vi "Game_Play.vi"(0 "State":T1={"Tick"=0, "Phase"=0, "PhaseTicks"=0, "Level"=1, "Room"=0, "X10"=0, "Y10"=0, "VY10"=0, "Mode"=0, "Facing"=0, "Run"=0, "Vert"=0, "StandY"=0, "EntryX10"=0, "EntryY10"=0, "EntryMode"=0, "Lives"=4, "Score"=0, "NextLife"=10000, "KeyR"=0, "KeyB"=0, "KeyY"=0, "Torch"=FALSE, "FloorPhase"=0, "Dead"=FALSE, "LevelStart"=FALSE, "Quit"=FALSE, "Sound"=0, "Seed"=12345, "DemoStep"=0, "Tiles"=[], "World"=[], "Enemies"=[], "Highscores"=[], "Name"=[0, 0, 0], "Cursor"=0}, 5 "Jump":bool, 11 "error in":errorcluster) -> (4 "State out":T1={"Tick"=0, "Phase"=0, "PhaseTicks"=0, "Level"=1, "Room"=0, "X10"=0, "Y10"=0, "VY10"=0, "Mode"=0, "Facing"=0, "Run"=0, "Vert"=0, "StandY"=0, "EntryX10"=0, "EntryY10"=0, "EntryMode"=0, "Lives"=4, "Score"=0, "NextLife"=10000, "KeyR"=0, "KeyB"=0, "KeyY"=0, "Torch"=FALSE, "FloorPhase"=0, "Dead"=FALSE, "LevelStart"=FALSE, "Quit"=FALSE, "Sound"=0, "Seed"=12345, "DemoStep"=0, "Tiles"=[], "World"=[], "Enemies"=[], "Highscores"=[], "Name"=[0, 0, 0], "Cursor"=0}, 6 "Hit":bool, 8 "Died":bool, 15 "error out":errorcluster)   [LabVIEW 2020, in "GH_Engine.lvlib"]
doc: "One tick of play: rhythm of the vanishing floors (FloorPhase), Claude moves (Player_Move, jump sound), takes objects (Items_Collect), opens doors (Door_Open), enemies move (Enemies_Step), Hit_Check, room change (Room_Change) and an extra life every 10000 points (at most 7). Hit = an enemy touches Claude, Died = deadly fall."
uses:
  GH_Engine.lvlib
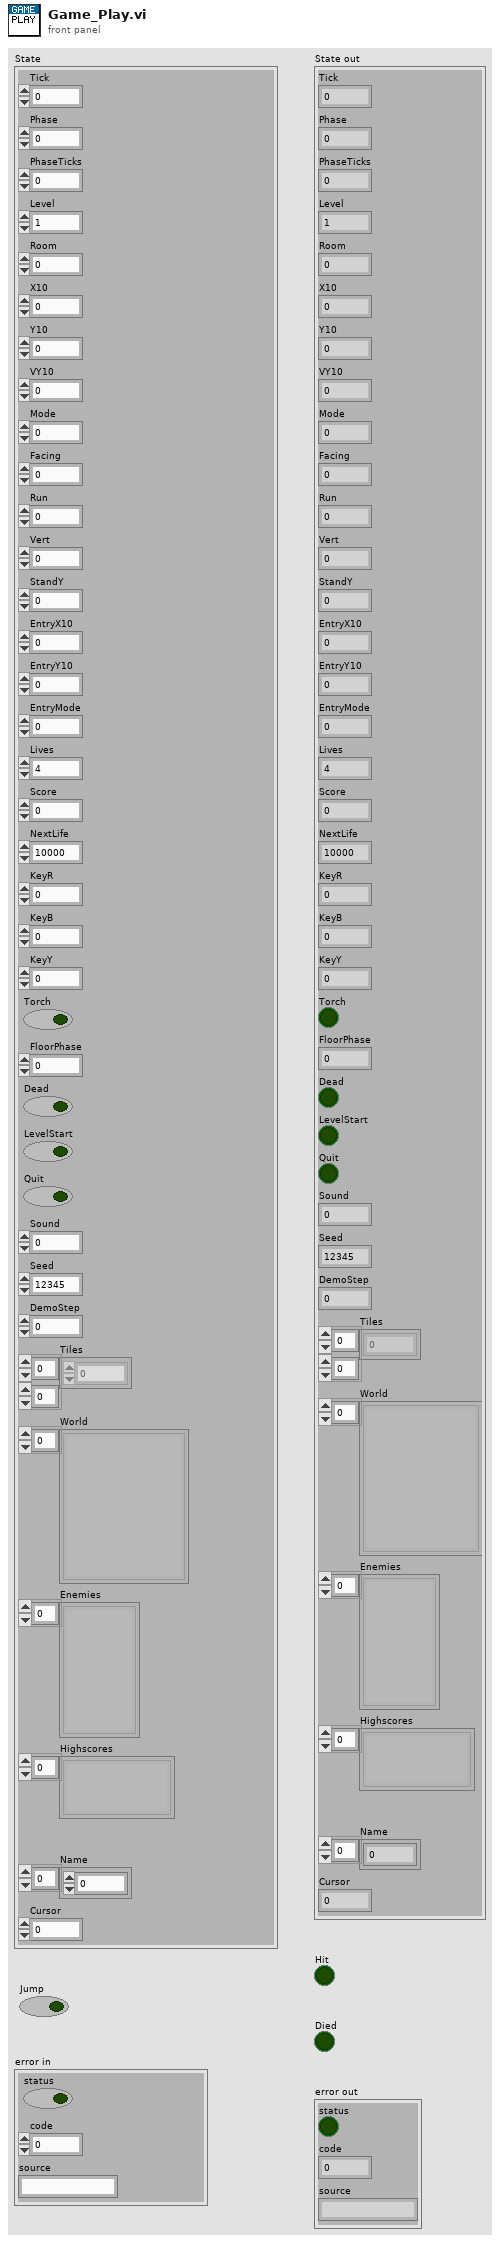
[diagram p1: front panel]
types:
  T1 = cluster{"Tick":u32, "Phase":i32, "PhaseTicks":i32, "Level":i32, "Room":i32, "X10":i32, "Y10":i32, "VY10":i32, "Mode":i32, "Facing":i32, "Run":i32, "Vert":i32, "StandY":i32, "EntryX10":i32, "EntryY10":i32, "EntryMode":i32, "Lives":i32, "Score":i32, "NextLife":i32, "KeyR":i32, "KeyB":i32, "KeyY":i32, "Torch":bool, "FloorPhase":i32, "Dead":bool, "LevelStart":bool, "Quit":bool, "Sound":i32, "Seed":u32, "DemoStep":i32, "Tiles":u8[][], "World":cluster{"ID":string, "Depth":i32, "Column":i32, "Tiles":u8[][]}[], "Enemies":cluster{"Kind":i32, "X10":i32, "Y10":i32, "Dir":i32, "Mode":i32}[], "Highscores":cluster{"Score":i32, "Name":string}[], "Name":i32[], "Cursor":i32}
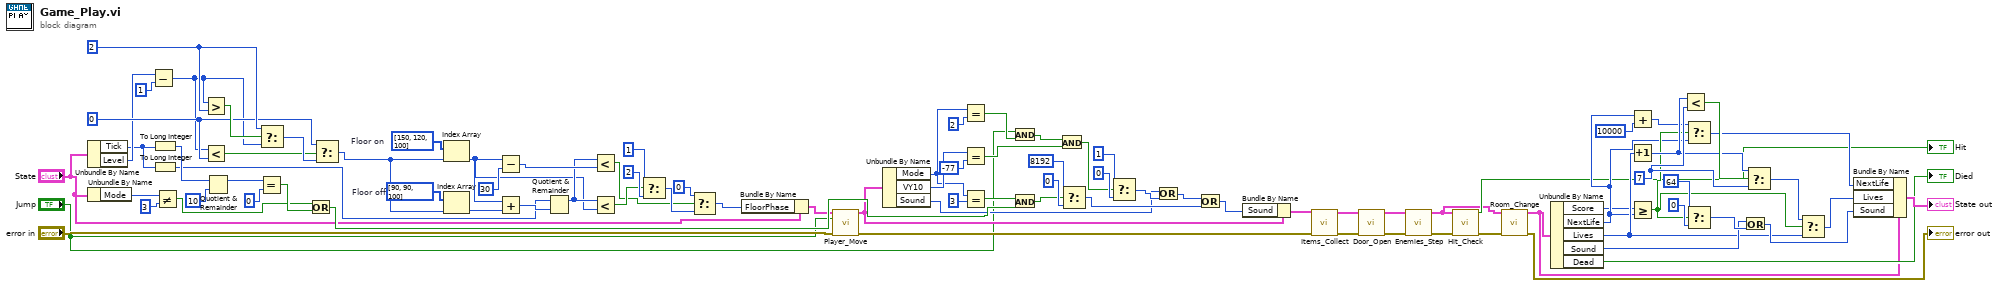
[diagram p0: block diagram]
diagram:
  w83 = 7
  w16 = i32[] [90, 90, 100]  # Floor off
  w14 = i32[] [150, 120, 100]  # Floor on
  w9 = 2
  w8 = 0
  n1 = Unbundle By Name("State") -> ("Tick"=w4:u32, "Level"=w5:i32)
  n2 = Unbundle By Name("State") -> ("Mode"=w42:i32)
  n3 = Subtract(x=w5, y=1) -> (x-y=w7:i32)
  n4 = To Long Integer(number=w4) -> (32bit integer=w47:i32)
  n5 = To Long Integer(number=w4) -> (32bit integer=w18:i32)
  n6 = Not Equal?(x=w42, y=3) -> (x != y?=w46:bool)
  n7 = Greater?(x=w7, y=w9) -> (0:w11:bool)
  n8 = Less?(x=w7, y=w8) -> (x < y?=w10:bool)
  n9 = Quotient & Remainder(x=w47, y=10) -> (x-y*floor(x/y)=w49:i32)  [unwired: 1 out]
  n10 = Equal?(x=w49, y=0) -> (x = y?=w51:bool)
  n11 = Select(t=w9, s=w11, f=w7) -> (s? t:f=w12:i32)
  n12 = Or(x=w46, y=w51) -> (x .or. y?=w52:bool)
  n13 = Select(t=w8, s=w10, f=w12) -> (s? t:f=w13:i32)
  n14 = Index Array(array=w14, index=w13) -> (element=w15:i32)
  n15 = Index Array(array=w16, index=w13) -> (element=w17:i32)
  n16 = Subtract(x=w15, y=30) -> (x-y=w22:i32)
  n17 = Add(x=w15, y=w17) -> (x+y=w19:i32)
  n18 = Quotient & Remainder(x=w18, y=w19) -> (x-y*floor(x/y)=w20:i32)  [unwired: 1 out]
  n19 = Less?(x=w20, y=w22) -> (x < y?=w23:bool)
  n20 = Less?(x=w20, y=w15) -> (x < y?=w25:bool)
  n21 = Select(t=1, s=w25, f=2) -> (s? t:f=w28:i32)
  n22 = Select(t=0, s=w23, f=w28) -> (s? t:f=w29:i32)
  n23 = Bundle By Name(cluster="State", "FloorPhase"=w29) -> (w30:T1)
  n24 = call "Player_Move.vi"("State"=w30, "Jump"="Jump", "error in"="error in") -> ("State out"=w31:T1, "error out"=w32:errorcluster)  [unwired: 11 in]
  n25 = Unbundle By Name(w31) -> ("Mode"=w33:i32, "VY10"=w34:i32, "Sound"=w35:i32)
  n26 = Equal?(x=w33, y=2) -> (x = y?=w37:bool)
  n27 = Equal?(x=w34, y=-77) -> (x = y?=w39:bool)
  n28 = Equal?(x=w33, y=3) -> (x = y?=w44:bool)
  n29 = And(x="Jump", y=w37) -> (x .and. y?=w40:bool)
  n30 = And(x=w44, y=w52) -> (x .and. y?=w53:bool)
  n31 = And(x=w40, y=w39) -> (x .and. y?=w41:bool)
  n32 = Select(t=8192, s=w53, f=0) -> (s? t:f=w60:i32)
  n33 = Select(t=1, s=w41, f=0) -> (s? t:f=w56:i32)
  n34 = Or(x=w35, y=w56) -> (x .or. y?=w57:i32)
  n35 = Or(x=w57, y=w60) -> (x .or. y?=w61:i32)
  n36 = Bundle By Name(cluster=w31, "Sound"=w61) -> (w62:T1)
  n37 = call "Items_Collect.vi"("State"=w62, "error in"=w32) -> ("State out"=w63:T1, "error out"=w64:errorcluster)  [unwired: 12 in]
  n38 = call "Door_Open.vi"("State"=w63, "error in"=w64) -> ("State out"=w65:T1, "error out"=w66:errorcluster)  [unwired: 11 in, 1 out]
  n39 = call "Enemies_Step.vi"("State"=w65, "error in"=w66) -> ("State out"=w67:T1, "error out"=w68:errorcluster)  [unwired: 12 in]
  n40 = call "Hit_Check.vi"("State"=w67, "error in"=w68) -> ("Hit"=→"Hit":bool, "error out"=w70:errorcluster)  [unwired: 12 in]
  n41 = call "Room_Change.vi"("State"=w67, "error in"=w70) -> ("State out"=w71:T1, "error out"=→"error out":errorcluster)  [unwired: 11 in, 1 out]
  n42 = Unbundle By Name(w71) -> ("Score"=w73:i32, "NextLife"=w74:i32, "Lives"=w75:i32, "Sound"=w76:i32, "Dead"=→"Died":bool)
  n43 = Add(x=w74, y=10000) -> (x+y=w80:i32)
  n44 = Increment(x=w75) -> (x+1=w82:i32)
  n45 = Greater Or Equal?(x=w73, y=w74) -> (x >= y?=w78:bool)
  n46 = Less?(x=w82, y=w83) -> (x < y?=w84:bool)
  n47 = Select(t=w80, s=w78, f=w74) -> (s? t:f=w81:i32)
  n48 = Select(t=64, s=w78, f=0) -> (s? t:f=w89:i32)
  n49 = Or(x=w76, y=w89) -> (x .or. y?=w90:i32)
  n50 = Select(t=w82, s=w84, f=w83) -> (s? t:f=w85:i32)
  n51 = Select(t=w85, s=w78, f=w75) -> (s? t:f=w86:i32)
  n52 = Bundle By Name(cluster=w71, "NextLife"=w81, "Lives"=w86, "Sound"=w90) -> (→"State out":T1)
